vi "Shift Zero (multiple).vi"(8 "error in (no error)":errorcluster, 10 "Zero x index":i32, 11 "XY-data":cluster{"X-array":dbl[], "Y-array":dbl[]}[](array[cluster])) -> (0 "error out":errorcluster, 3 "Shifted XY-data out":cluster{"X-array":dbl[], "Y-array":dbl[]}[](array[cluster]) {"Y-array" format="%.2p"; "X-array" format="%.2p"})   [LabVIEW 2019, in "xy_utilities.lvlib"]
doc: "Shift the zero value of the x array by giving a new fractional x index.\n\nWire data to the data input to determine the polymorphic instance to use or manually select the instance."
uses:
  xy_utilities.lvlib
  <vilib>/gmath/interp.llb/Interpolate 1D.vi
  <vilib>/Utility/error.llb/Error Cluster From Error Code.vi
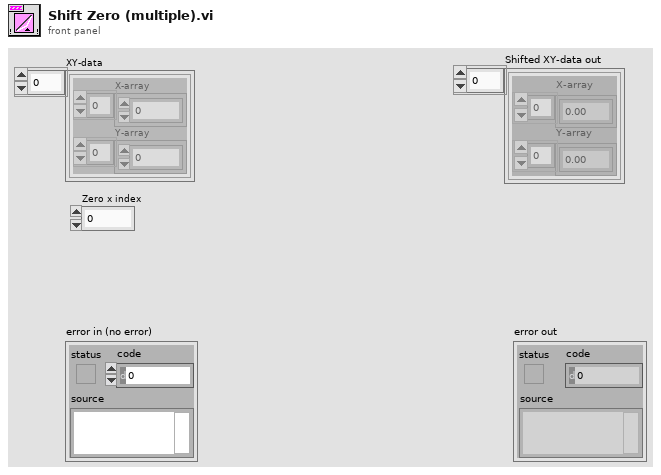
[diagram p1: front panel]
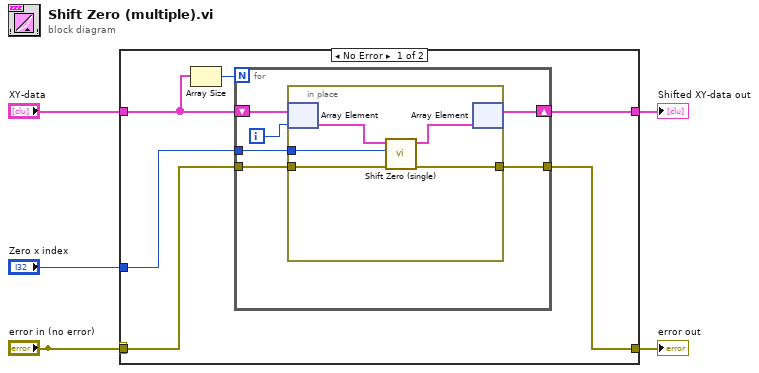
[diagram p0: block diagram]
diagram:
  n1 = case shown="No Error" "error in (no error)" {
    selector: "error in (no error)" -> [_ w24]
    tunnel: [w8 w24] -> w5
    tunnel: "XY-data" -> [w6 w23]
    tunnel: [w9 w23] -> w1
    tunnel: "Zero x index" -> [w10 _]
    tunnel: "error in (no error)" -> [w11 _]
    frame No Error {
      n2 = Array Size(array=w6) -> (size(s)=w7:i32)
      n3 = for {
        N: w7 -> [_]
        tunnel: w11 -> [w17]
        tunnel: w10 -> [w16]
        tunnel: [w15] -> w8
        shift-right: [w12] -> w9
        shift-left: w6 -> [w14]
        i -> [w13]
        n4 = in-place {
          in-place-border: w17 -> [w22]
          in-place-border: w16 -> [w21]
          in-place-border: [w20] -> w15
          n5 = in-place-array #1(w14, w13) -> (w18:cluster{"X-array":dbl[], "Y-array":dbl[]})
          n6 = call "Shift Zero (single).vi"("error in (no error)"=w22, "Zero x index"=w21, "XY-data"=w18) -> ("error out"=w20:errorcluster, "Shifted XY-data out"=w19:cluster{"X-array":dbl[], "Y-array":dbl[]})  [unwired: 7 in]
          n7 = in-place-array #1(w19) -> (w12:cluster{"X-array":dbl[], "Y-array":dbl[]}[])  [unwired: 1 out]
        }
      }
    }
    frame Error {
    }
  }
  "error out" <- w5
  "Shifted XY-data out" <- w1
